vi "PicoScope5000aGetStreamingValues.vi"(10 "handle in":i16, 11 "error in":errorcluster) -> (0 "Start Index in Driver Buffer":u32, 1 "Trigger":cluster{bool, "triggeredAt (Total samples)":u32}, 2 "handle out":i16, 3 "error out":errorcluster, 4 "Number of Samples":u32, 5 "ready":i16, 6 "Auto Stopped":bool)   [LabVIEW 2010]
doc: "This VI is used in streaming mode to get the latest values from the driver. It should be called in a loop after the oscilloscope has been set up using PicoScope5000aSettings.vi and streaming has been started by calling PicoScope5000aStartStreaming.vi. The VI outputs the number of samples available and the start index of these samples in the array output by PicoScope5000aStartStreaming.vi."
uses:
  ps5000aWrap.dll
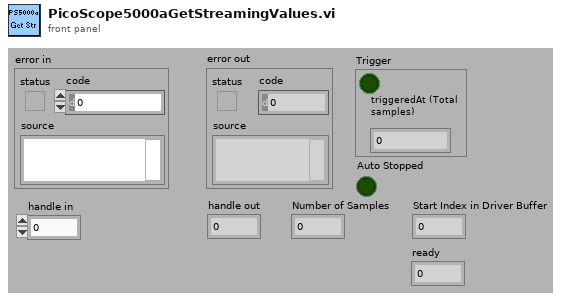
[diagram p1: front panel]
types:
  T1 = cluster{"status":bool, "code":u32, "source":string}
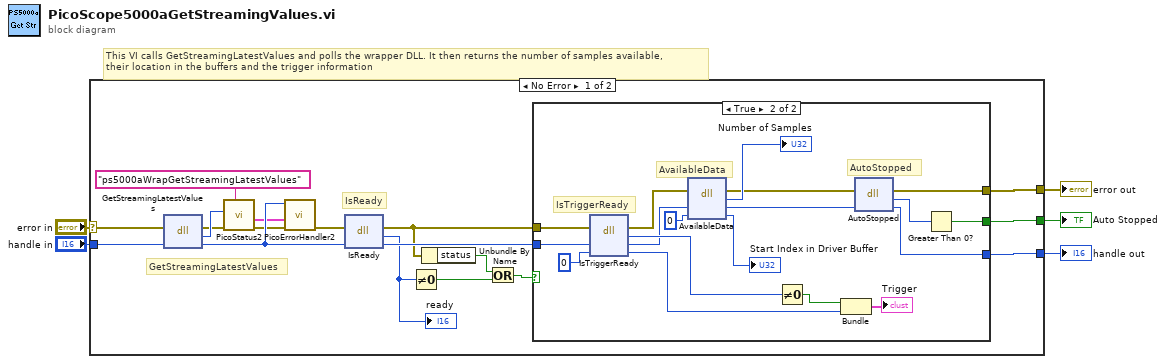
[diagram p0: block diagram]
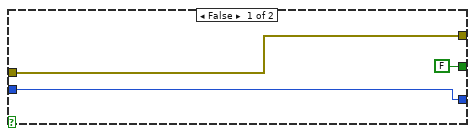
[diagram p2: hidden frame]
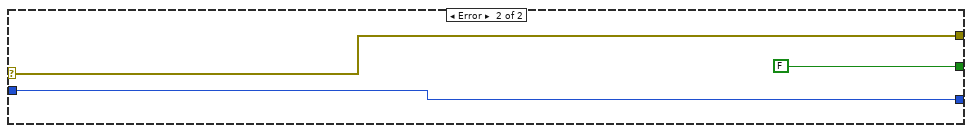
[diagram p3: hidden frame]
diagram:
  # "This VI calls GetStreamingLatestValues and polls the wrapper DLL. It then returns the number of samples available, \ntheir location in the buffers and the trigger information"
  n1 = case shown="No Error" "error in" {
    selector: "error in" -> [w18 w47]
    tunnel: [w23 w47] -> w4
    tunnel: "handle in" -> [w17 w46]
    tunnel: [w20 w46] -> w2
    tunnel: [w19 FALSE] -> w1
    frame No Error {
      # "GetStreamingLatestValues"
      # "IsReady"
      n2 = dll-call lib="ps5000aWrap.dll" fn="GetStreamingLatestValues" ("PS5000.dll:_ps5000SetDataBuffer@16")(error in=w18, "handle"=w17) -> (error out=w12:errorcluster, "PICO_STATUS"=w13:u32, "handle"=w10:i16)  [unwired: 2 in, 1 out]
      n3 = call "PicoStatus2.vi"("PICO source"="ps5000aWrapGetStreamingLatestValues" ("source"), "Error in"=w12, "PICO STATUS"=w13) -> ("error out"=w9:errorcluster, "PICO_STATUS out"=w6:T1)  [unwired: 5 in]
      n4 = call "PicoErrorHandler2.vi"("error in (no error)"=w9, "PICO_STATUS in"=w6, "handle In"=w10) -> ("error out"=w8:errorcluster)  [unwired: 8 in]
      n5 = dll-call lib="ps5000aWrap.dll" fn="IsReady" ("PS5000.dll:_ps5000SetDataBuffer@16")(error in=w8, "handle"=w10) -> (error out=w21:errorcluster, "ready"=w16:i16, "handle"=w22:i16)  [unwired: 2 in, 1 out]
      "ready" <- w16
      n6 = Not Equal To 0?(x=w16) -> (x != 0?=w14:bool)
      n7 = Unbundle By Name(w21) -> ("status"=w15:bool)
      n8 = Or(x=w15, y=w14) -> (x .or. y?=w7:bool)
      n9 = case shown="True" w7 {
        tunnel: [w26 w27] -> w23
        tunnel: w22 -> [w25 w43]
        tunnel: w21 -> [w26 w35]
        tunnel: [w25 w32] -> w20
        tunnel: [FALSE w30] -> w19
        frame False {
        }
        frame True {
          # "AutoStopped"
          # "AvailableData"
          # "IsTriggerReady"
          n10 = dll-call lib="ps5000aWrap.dll" fn="IsTriggerReady" ("PS5000.dll:_ps5000SetDataBuffer@16")(error in=w35, "handle"=w43, "triggeredAt"=u32 0) -> (error out=w39:errorcluster, "triggered"=w42:i16, "handle"=w38:i16, "triggeredAt"=w28:u32)  [unwired: 2 in, 1 out]
          n11 = dll-call lib="ps5000aWrap.dll" fn="AvailableData" ("PS5000.dll:_ps5000Stop@4")(error in=w39, "handle"=w38, "startIndex"=u32 0) -> (error out=w34:errorcluster, "numSamples"=→"Number of Samples":u32, "handle"=w33:i16, "startIndex"=→"Start Index in Driver Buffer":u32)  [unwired: 2 in, 1 out]
          n12 = Not Equal To 0?(x=w42) -> (x != 0?=w41:bool)
          n13 = Bundle(w41, "triggeredAt"=w28) -> (→"Trigger":cluster{bool, "triggeredAt":u32})  [unwired: 1 in]
          n14 = dll-call lib="ps5000aWrap.dll" fn="AutoStopped"(error in=w34, "handle"=w33) -> (error out=w27:errorcluster, "autoStopped"=w31:i16, "handle"=w32:i16)  [unwired: 2 in, 1 out]
          n15 = Greater Than 0?(x=w31) -> (x > 0?=w30:bool)
        }
      }
    }
    frame Error {
    }
  }
  "error out" <- w4
  "handle out" <- w2
  "Auto Stopped" <- w1
